vi "Read Time Sync.vi"(8 "error in (no error)":errorcluster, 11 "RT Data Cluster in":T1={"Timekeeper hdl"="", "clkDisc session"=variant, "Compiled Data"={"SyncMod?"=FALSE, "SyncMod"="", "ConnectionSettings"={"Mode"=enum."Generate sample clock", "pxitrig"=FALSE, "pfi0"=FALSE, "pfi1"=FALSE, "pfi2"=FALSE, "External Pin"=enum."PFI0", "Routes"=[]}, "TimeKeeper"="", "ScanOffset(%)"=0.0, "StartDelay(s)"=0, "Time Ref Settings"={"Time Reference"=enum."GPS", "Priority 1"=0, "Priority 2"=0, "IRIG type"=enum."IRIGB AM", "Terminal"="", "PPSSetTime"=FALSE, "Start Time"=timestamp(0 s since 1904-01-01)}, "FIFO Locations"={"BoardTime"=[], "Status"=[]}}, "OutputsData"=[], "OutputsFIFO"=refnum, "Scan Period"=0, "Timekeeper type"=enum."6683", "SyncMod type"=enum."6683", "SyncMod hdl"="", "Custom Device Name"=""} {"Compiled Data"."Time Ref Settings"."Priority 2" min=0 max=255; "Compiled Data"."Time Ref Settings"."Priority 1" min=0 max=255}) -> (0 "error out":errorcluster, 3 "RT Data Cluster out":T1={"Timekeeper hdl"="", "clkDisc session"=variant, "Compiled Data"={"SyncMod?"=FALSE, "SyncMod"="", "ConnectionSettings"={"Mode"=enum."Generate sample clock", "pxitrig"=FALSE, "pfi0"=FALSE, "pfi1"=FALSE, "pfi2"=FALSE, "External Pin"=enum."PFI0", "Routes"=[]}, "TimeKeeper"="", "ScanOffset(%)"=0.0, "StartDelay(s)"=0, "Time Ref Settings"={"Time Reference"=enum."GPS", "Priority 1"=0, "Priority 2"=0, "IRIG type"=enum."IRIGB AM", "Terminal"="", "PPSSetTime"=FALSE, "Start Time"=timestamp(0 s since 1904-01-01)}, "FIFO Locations"={"BoardTime"=[], "Status"=[]}}, "OutputsData"=[], "OutputsFIFO"=refnum, "Scan Period"=0, "Timekeeper type"=enum."6683", "SyncMod type"=enum."6683", "SyncMod hdl"="", "Custom Device Name"=""} {"Compiled Data"."Time Ref Settings"."Priority 2" min=0 max=255; "Compiled Data"."Time Ref Settings"."Priority 1" min=0 max=255})   [LabVIEW 2020, in "NI Synchronization Engine.lvlib"]
uses:
  NI Synchronization Engine.lvlib
  <resource>/objmgr/timeSync.rc
  mdevClkDisc.llb/_clkDisc_session.ctl
  Shared/Route.ctl
  Shared/NI Synchronization Shared.lvlib
  Shared/Routes.ctl
  Shared/External Pin.ctl
  Shared/Mode.ctl
  Shared/Connection Settings.ctl
  Shared/IRIG Type.ctl
  Shared/Time Ref Settings.ctl
  Shared/Compiled Data.ctl
  RT Data Cluster.ctl
  Shared/Time Reference.ctl
  timekeeper type.ctl
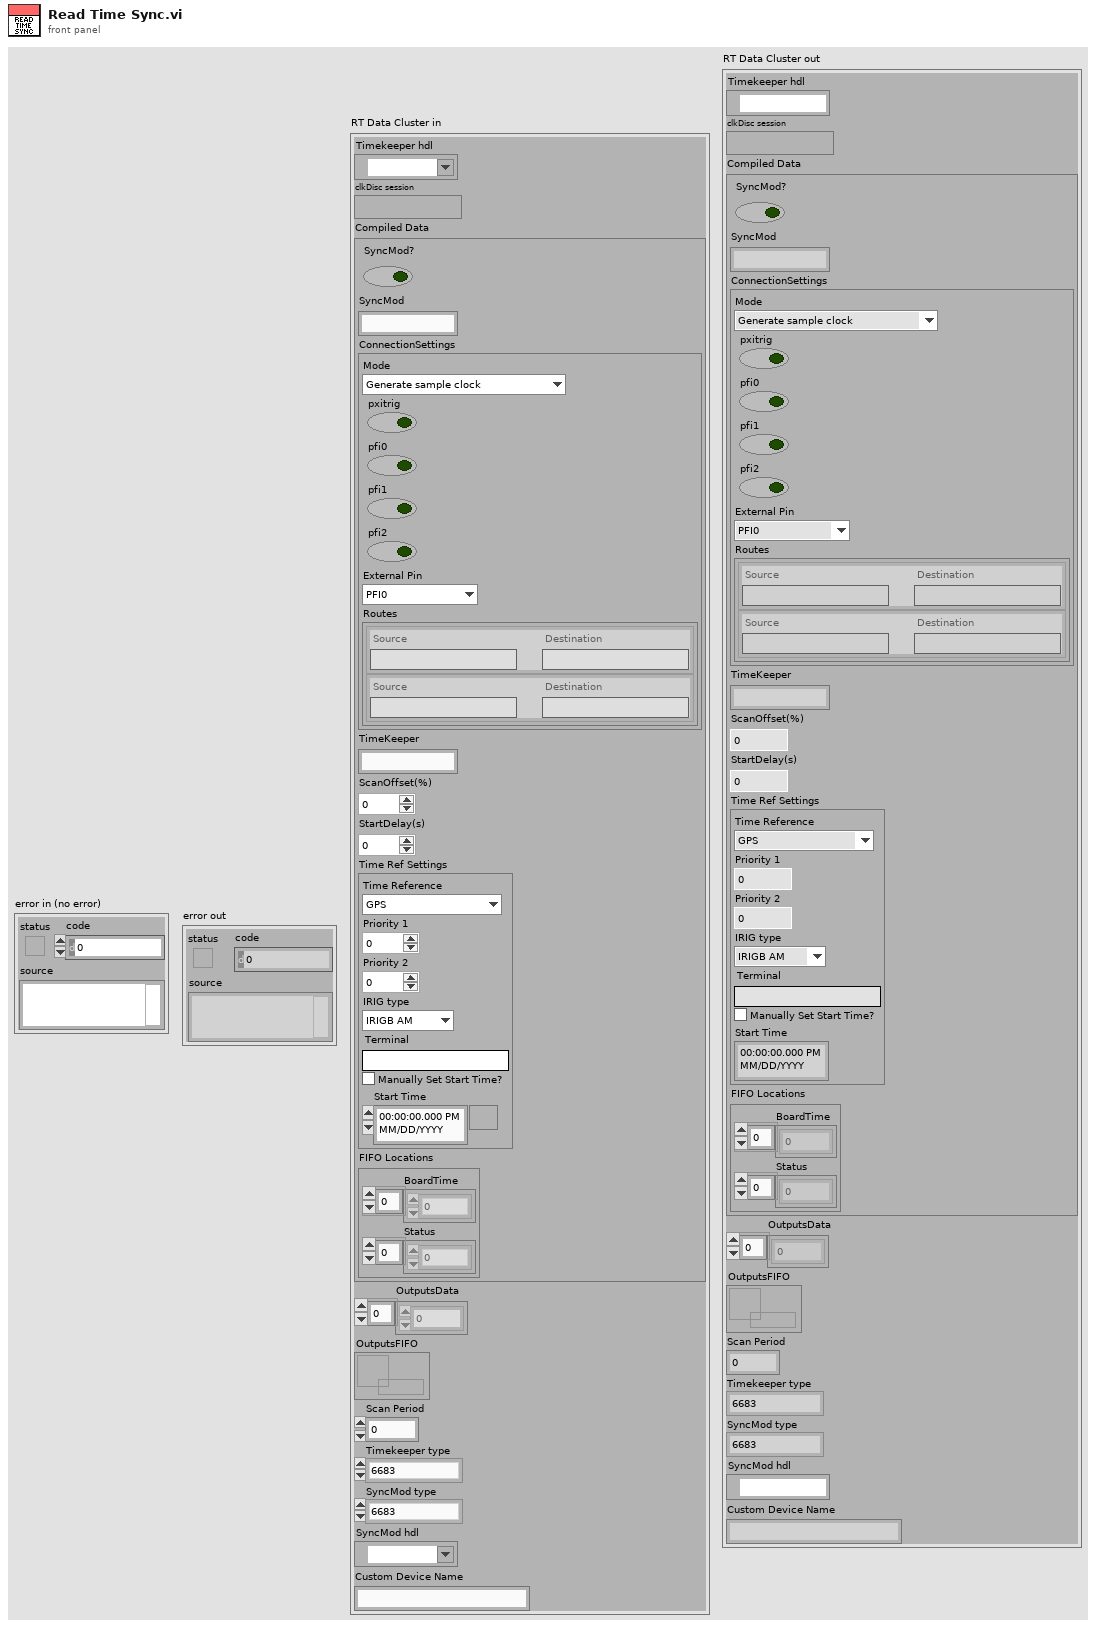
[diagram p1: front panel]
types:
  T1 = typedef "NI Synchronization Engine.lvlib/RT Data Cluster.ctl" = cluster{"Timekeeper hdl":refnum<k15>, "clkDisc session":T2, "Compiled Data":T3, "OutputsData":dbl[], "OutputsFIFO":refnum<k33>, "Scan Period":u32, "Timekeeper type":T12, "SyncMod type":T12, "SyncMod hdl":refnum<k15>, "Custom Device Name":string}
  T2 = typedef "_clkDisc_session.ctl" = variant
  T3 = typedef "NI Synchronization Shared.lvlib/Compiled Data.ctl" = cluster{"SyncMod?":bool, "SyncMod":string, "ConnectionSettings":T4, "TimeKeeper":string, "ScanOffset(%)":dbl, "StartDelay(s)":u16, "Time Ref Settings":T9, "FIFO Locations":cluster{"BoardTime":i32[], "Status":i32[]}}
  T4 = typedef "NI Synchronization Shared.lvlib/Connection Settings.ctl" = cluster{"Mode":T5, "pxitrig":bool, "pfi0":bool, "pfi1":bool, "pfi2":bool, "External Pin":T6, "Routes":T7}
  T5 = typedef "NI Synchronization Shared.lvlib/Mode.ctl" = enum16{"Generate sample clock", "Route sample clock out of chassis", "Route sample clock into chassis", "Custom routes"}
  T6 = typedef "NI Synchronization Shared.lvlib/External Pin.ctl" = enum16{"PFI0", "PFI1", "PFI2"}
  T7 = typedef "NI Synchronization Shared.lvlib/Routes.ctl" = T8[]
  T8 = typedef "NI Synchronization Shared.lvlib/Route.ctl" = cluster{"Source":string, "Destination":string}
  T9 = typedef "NI Synchronization Shared.lvlib/Time Ref Settings.ctl" = cluster{"Time Reference":T10, "Priority 1":i32, "Priority 2":i32, "IRIG type":T11, "Terminal":string, "PPSSetTime":bool, "Start Time":timestamp}
  T10 = typedef "NI Synchronization Shared.lvlib/Time Reference.ctl" = enum16{"GPS", "IRIG", "PPS", "1588 Ordinary Clock", "802.1AS", "PXI Chassis Clock", "Free Running (Internal)"}
  T11 = typedef "NI Synchronization Shared.lvlib/IRIG Type.ctl" = enum16{"IRIGB DC", "IRIGB AM"}
  T12 = typedef "NI Synchronization Engine.lvlib/timekeeper type.ctl" = enum16{"6683", "6683H", "6682", "6682H", "non-timekeeper", "timekeeper"}
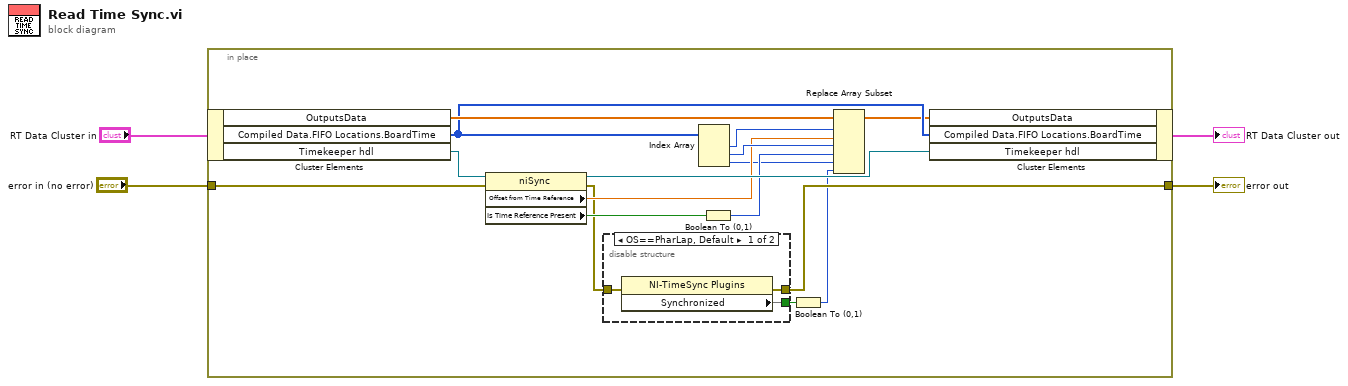
[diagram p0: block diagram]
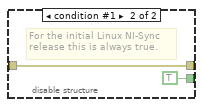
[diagram p2: hidden frame]
diagram:
  n1 = in-place {
    in-place-border: "error in (no error)" -> [w17]
    in-place-border: [w8] -> w2
    n2 = in-place-cluster #1("RT Data Cluster in") -> ("OutputsData"=w20:dbl[], "Compiled Data.FIFO Locations.BoardTime"=w19:i32[], "Timekeeper hdl"=w18:refnum<k15>)
    n3 = property class="niSync"(reference=w18, error in=w17) -> (reference out=w14:refnum<k15>, error out=w9:errorcluster, "Offset from Time Reference"=w12:dbl, "Is Time Reference Present"=w16:bool)
    n4 = disable-structure shown="OS==PharLap, Default" {
      disable-tunnel: w9 -> [w23 w25]
      disable-tunnel: [w22 w25] -> w8
      disable-tunnel: [w21 TRUE ("Synchronized")] -> w6
      frame condition #0 (active) {
        n5 = property class="NI-TimeSync Plugins"(error in=w23) -> (error out=w22:errorcluster, "Synchronized"=w21)  [unwired: 1 in, 1 out]
      }
      frame condition #1 {
        # "For the initial Linux NI-Sync\nrelease this is always true."
      }
    }
    n6 = Index Array(array=w19) -> (element #1=w7:i32, element #2=w13:i32, element #3=w10:i32)  [unwired: 3 in]
    n7 = Boolean To (0,1)(Boolean=w16) -> (0, 1=w11:i16)
    n8 = Boolean To (0,1)(Boolean=w6) -> (0, 1=w5:i16)
    n9 = Replace Array Subset(array=w20, new element #1=w12, index #1=w7, new element #2=w11, index #2=w13, new element #3=w5, index #3=w10) -> (w15:dbl[])
    n10 = in-place-cluster #1("OutputsData"=w15, "Compiled Data.FIFO Locations.BoardTime"=w19, "Timekeeper hdl"=w14) -> (→"RT Data Cluster out":T1)
  }
  "error out" <- w2
